vi "Native_AddEventFrame_v2.vi"() -> ()   [LabVIEW 2024]
panel:
  out "error out":errorcluster caption="错误输出"
  out "frame_id":u32
  in  "frame_id type":u32
  in  "reference_frame_index":u32
  in  "event_id":u32
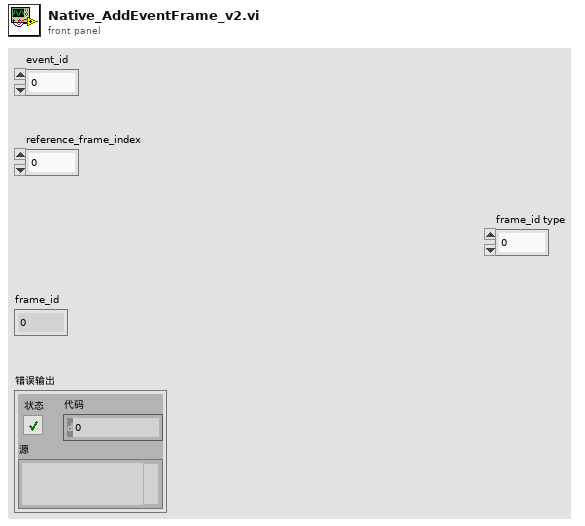
[diagram p1: front panel]
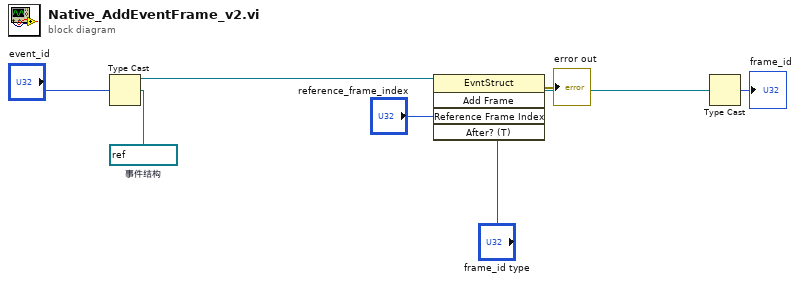
[diagram p0: block diagram]
diagram:
  w7 = refnum<vi> refnum  # 事件结构
  n1 = Type Cast ("强制类型转换")(type=w7, x="event_id") -> (*(type *) &x=w6:refnum<vi>)
  n2 = invoke class="EvntStruct" method="Add Frame"(reference=w6, "Reference Frame Index"="reference_frame_index") -> (error out=→"error out":errorcluster, "Add Frame"=w4:refnum<vi>)  [unwired: 3 in, 3 out]
  n3 = Type Cast ("强制类型转换")(type="frame_id type", x=w4) -> (*(type *) &x=→"frame_id":u32)
